vi "Set Engine Scan Rate.vi"(8 "error in (no error)":errorcluster, 9 "Configure Scan Engine":bool, 10 "scan period (uSec)":u32=10000, 11 "references in":T1) -> (0 "error out":errorcluster, 3 "references out":T1)   [LabVIEW 2015, in "Scan Engine editor node.lvclass"]
uses:
  Scan Engine editor node.lvclass
  <vilib>/NI/DCAF/Tag Editor Core/Table API/Table Manager/object ref.ctl
  <vilib>/NI/DCAF/Tag Editor Core/Configuration Editor/Classes/Engine Parent/Engine Parent Editor Node.lvclass
  <vilib>/NI/DCAF/Tag Editor Core/Configuration Editor/Classes/Module editor node/module editor node.lvclass
  configuration/Scan Engine configuration.lvclass
  <vilib>/NI/DCAF/Tag Editor Core/Configuration Editor/Classes/Module editor node/Read Module Configuration.vi
  <vilib>/NI/DCAF/Tag Editor Core/Configuration Editor/Classes/Module editor node/Write Module Configuration.vi
  <vilib>/NI/Tag Bus Module Framework/module configuration/TBM module configuration.lvclass
  <vilib>/NI/DCAF/Tag Editor Core/Table API/Table Manager/Table Manager.lvclass
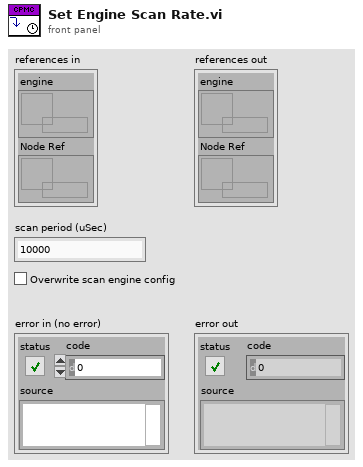
[diagram p1: front panel]
types:
  T1 = typedef "Table Manager.lvlib/Table Manager.lvclass/object ref.ctl" = cluster{"engine":refnum<data-value>, "Node Ref":refnum<data-value>}
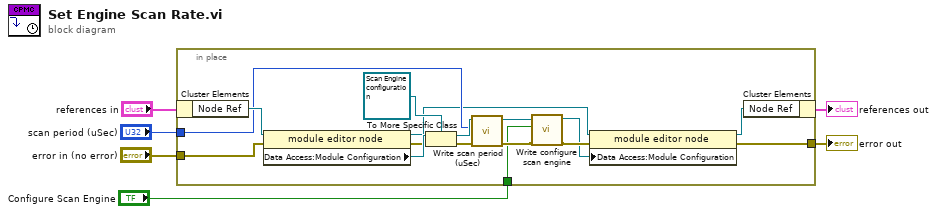
[diagram p0: block diagram]
diagram:
  n1 = in-place {
    in-place-border: "scan period (uSec)" -> [w18]
    in-place-border: "error in (no error)" -> [w15]
    in-place-border: [w12] -> w3
    in-place-border: "Configure Scan Engine" -> [w7]
    n2 = in-place-cluster #1("references in") -> ("Node Ref"=w21:refnum<data-value>)
    n3 = property class="module editor node"(reference=w21, error in=w15) -> (reference out=w17:refnum<data-value>, error out=w14:errorcluster, "Data Access:Module Configuration"=w20:refnum<class "TBM module configuration.lvclass">)
    n4 = To More Specific Class(target class=refnum<class "Scan Engine configuration.lvclass"> refnum ("Scan Engine configuration"), reference=w20, error in=w14) -> (specific class reference=w19:refnum<class "Scan Engine configuration.lvclass">, error out=w13:errorcluster)
    n5 = call-dynamic "Write scan period (uSec).vi"("error in (no error)"=w13, "scan period (uSec)"=w18, "Scan Engine configuration1 in"=w19) -> ("error out"=w11:errorcluster, "Scan Engine configuration1 out"=w9:refnum<class "Scan Engine configuration.lvclass">)  [unwired: 7 in]
    n6 = call-dynamic "Write configure scan engine.vi"("error in (no error)"=w11, "configure scan engine"=w7, "Scan Engine configuration1 in"=w9) -> ("error out"=w10:errorcluster, "Scan Engine configuration1 out"=w8:refnum<class "Scan Engine configuration.lvclass">)  [unwired: 7 in]
    n7 = property class="module editor node"(reference=w17, error in=w10, "Data Access:Module Configuration"=w8) -> (reference out=w16:refnum<data-value>, error out=w12:errorcluster)
    n8 = in-place-cluster #1("Node Ref"=w16) -> (→"references out":T1)
  }
  "error out" <- w3
